vi "kernel32 GetCurrentThreadId.vi"(11 "error in":errorcluster) -> (4 "thread ID":u32, 15 "error out":errorcluster)   [LabVIEW 2020, in "RemoteVI.lvlib"]
doc: "Returns the identifier of the calling thread through kernel32.dll GetCurrentThreadId (stdcall, called in LabVIEW's UI thread, so it is the UI thread's identifier - the thread whose key state user32 SetKeyboardState.vi writes). When error in carries an error the DLL is not called. Generated by scripts\\Build Win32 Wrappers.vi - do not edit by hand, rebuild it."
uses:
  RemoteVI.lvlib
  kernel32.dll
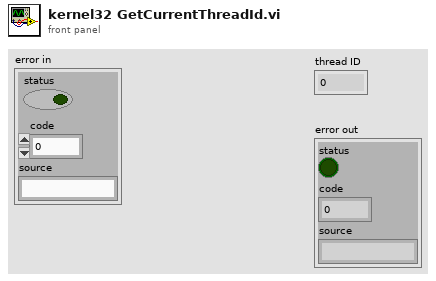
[diagram p1: front panel]
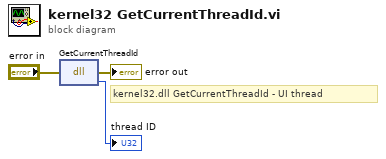
[diagram p0: block diagram]
diagram:
  # "kernel32.dll GetCurrentThreadId - UI thread"
  n1 = dll-call lib="kernel32.dll" fn="GetCurrentThreadId"(error in="error in") -> (error out=→"error out":errorcluster, →"thread ID":u32)  [unwired: 2 in, 1 out]
